vi "时间转Excel数字.vi"(10 "温湿度采集时刻":timestamp) -> (2 "数值":dbl)   [LabVIEW 2026, in "UI-湿度测量.lvlib" / "Logging.lvlib"]
uses:
  Logging.lvlib
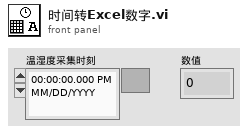
[diagram p1: front panel]
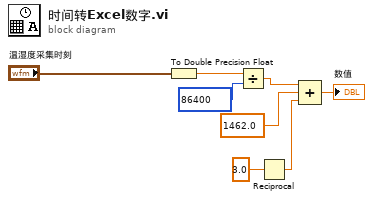
[diagram p0: block diagram]
diagram:
  n1 = To Double Precision Float(number="温湿度采集时刻") -> (double precision float=w5:dbl)
  n2 = Divide(x=w5, y=86400) -> (x/y=w7:dbl)
  n3 = Reciprocal(x=3.0) -> (1/x=w3:dbl)
  n4 = Compound Arithmetic op=ADD(w7, 1462.0 ("x/y"), w3) -> (→"数值":dbl)
